vi "Configure RemIO Module Core.vi"(8 "error in (no error)":errorcluster, 9 "module slot index":u8=1, 10 "Slave Ref In":refnum<k21>, 11 "11115 in":refnum<class "11115.lvclass">) -> (0 "error out":errorcluster, 1 "negative confirmation":T1 {"additional error code" format="%.0x"; "error code" format="%.0x"}, 2 "Slave Ref Out":refnum<k21>, 3 "11115 out":refnum<class "11115.lvclass">, 5 "SDO abort code":u32 format="%.0x")   [LabVIEW 2020, in "Modules.lvlib" / "11115.lvclass"]
uses:
  11115.lvclass
  <vilib>/indcomecat/Remote IO/typedefs/negative confirmation.ctl
  11115.lvclass/11115.ctl
  11d4ca15-a2fd-4149-8101-d2ecbe0d37f2.vi
  RemIO Module/Get RemIO Library Path.vi
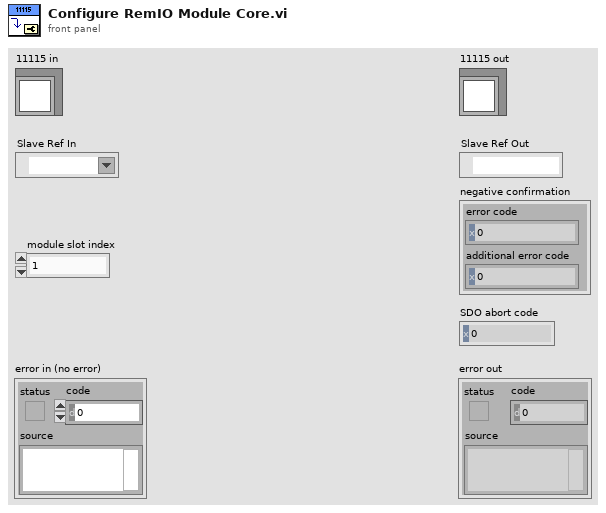
[diagram p1: front panel]
types:
  T1 = typedef "negative confirmation.ctl" = cluster{"error code":u16, "additional error code":u16}
  T2 = typedef "NI ECAT Remote IO.lvlib/channel number REM-11115.ctl" = u8
  T3 = typedef "NI ECAT Remote IO.lvlib/output range REM-11115.ctl" = u8
  T4 = cluster{"channel number":T2, "output range":T3}[]
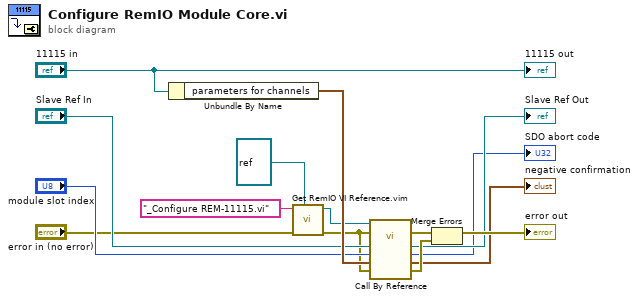
[diagram p0: block diagram]
diagram:
  n1 = Unbundle By Name("11115 in") -> ("parameters for channels"=w11:T4)
  n2 = call "Get RemIO VI Reference.vim"("name or relative path"="_Configure REM-11115.vi", "error in (no error)"="error in (no error)", "type specifier VI Refnum (for type only)"=refnum<vi> refnum) -> ("vi reference"=w1:refnum<vi>, "error out"=w4:errorcluster)  [unwired: 6 in]
  n3 = call-by-ref "?"(reference=w1, error in=w4, 8:"error in (no error)"=w4, "parameters for channels"=w11, "module slot index"="module slot index", "slave reference in"="Slave Ref In") -> (error out=w13:errorcluster, 0:"error out"=w14:errorcluster, "negative confirmation"=→"negative confirmation":T1, "SDO abort code"=→"SDO abort code":u32, "slave reference out"=→"Slave Ref Out":refnum<k21>)  [unwired: 4 in, 1 out]
  n4 = Merge Errors(w13, w14) -> (→"error out":errorcluster)
  "11115 out" <- "11115 in"
